vi "Acquisition.vi"(7 "CSM Name":string="CSM-Module") -> ()   [LabVIEW 2026, in "UI-湿度测量.lvlib" / "Acquisition.lvlib"]
doc: "------------- lvcsm -------------\n[CSMStates]\nItem 0 = \"Idle\"\nItem 1 = \"CSM Documentation\"\nItem 2 = \"VI Reference\"\nItem 3 = \"Error Handler\"\nItem 4 = \"Critical Error\"\nItem 5 = \"Target Timeout Error\"\nItem 6 = \"Target Error\"\nItem 7 = \"Async Response\"\nItem 8 = \"Response\"\nItem 9 = \"Async Message Posted\"\nItem 10 = \"Initialize Core Data\"\nItem 11 = \"Exit\"\nItem 12 = \"Data: Initialize\"\nItem 13 = \"Data: Update Indicators\"\nItem 14 = \"Data: Cleanup\"\nItem 15 = \"Macro: Initialize\"\nItem 16 = \"Macro: Exit\"\nItem 17 = \"API: API1\"\nItem 18 = \"API: Start\"\nItem 19 = \"API: Stop\"\nItem 20 = \"DAQ: Initialize\"\nItem 21 = \"DAQ: Acquisite\"\nItem 22 = \"DAQ: Stop\"\nItem 23 = \"DAQ: Close\"\nItem 24 = \"Continuous Check\"\nItem 25 = \"Break Continuous\"\n\n[CSMStatus]\nItem 0 = \"Error Occurred@Error Handler\"\nItem 1 = \"Acquired Data@DAQ: Acquisite\""
uses:
  Acquisition.lvlib
  Supports/Sample Settings.ctl
  Supports/Acquiring States.ctl
  Data ColndSave/Supports/Time and Data.ctl
  13cb97ba-6c5d-4c34-b6e1-a30149b67593.vi
  743750a1-4525-4ef4-b560-e15176358fb5.vi
  0392c9e0-fa12-4efc-b600-051e1718204e.vi
  <userlib>/_NEVSTOP/Communicable State Machine(CSM)/AdvanceAPI/CSM - Revert Arguments-Safe String.vi
  <userlib>/_NEVSTOP/Communicable State Machine(CSM)/_Shared/Trim Single-line Text.vi
  <userlib>/_NEVSTOP/Communicable State Machine(CSM)/AdvanceAPI/CSM - Make String Arguments Safe.vi
  <userlib>/_NEVSTOP/Communicable State Machine(CSM)/AdvanceAPI/CSM - Break Down Multiple States String.vi
  <userlib>/_NEVSTOP/Communicable State Machine(CSM)/AdvanceAPI/CSM - Compact Multiple States.vi
  <userlib>/_NEVSTOP/Communicable State Machine(CSM)/AdvanceAPI/CSM - Keywords.vi
  <userlib>/_NEVSTOP/Communicable State Machine(CSM)/addons/API-String-Arugments-Support/_Support/Convert API String Arguments to Data(variant).vi
  <vilib>/Instr/_visa.llb/VISA Configure Serial Port (Instr).vi
  <userlib>/_NEVSTOP/Communicable State Machine(CSM)/addons/MassData-Parameter/_support/FGV-MassData(lvlibp).vi
  <userlib>/_NEVSTOP/Communicable State Machine(CSM)/Communicable State Machine.lvlib
  <userlib>/_NEVSTOP/Communicable State Machine(CSM)/addons/Loop-Support/CSM Loop Support.lvlib
  Data ColndSave/Data Collection and Save.lvlib
panel:
  out "Error Occurred":errorcluster
  out "State History":string
  in  "Exit":bool
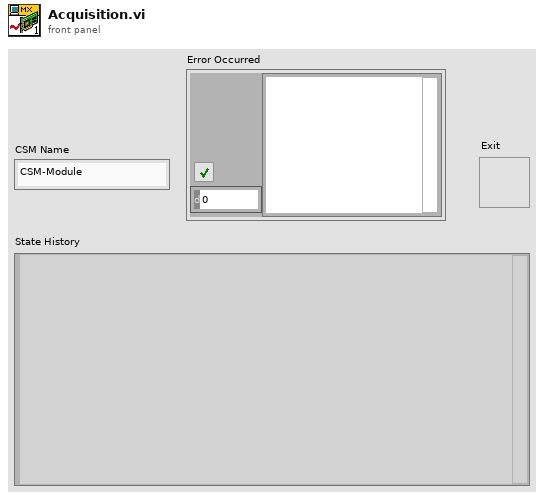
[diagram p1: front panel]
types:
  T1 = enum32{"Invalid", "Standard", "Closed", "Hidden", "Minimized", "Maximized"}
  T2 = enum32{"invalid app kind", "Development System", "Run Time System", "Student Edition", "Embedded LabVIEW", "Evaluation", "Custom"}
  T3 = typedef "UI-湿度测量.lvlib/Acquisition.lvlib/Acquiring States.ctl" = enum16{"Idle", "Acquiring", "Error"}
  T4 = cluster{"波特率":u32, "数据位":u16, "校验":enum16{"None", "Odd", "Even", "Mark", "Space"}, "停止位":u16, "流控制":u16}
  T5 = typedef "Communicable State Machine.lvlib/_CSM_Response Source Message.ctl" = cluster{"‘State":string, "’Arguments":string, "’Error":errorcluster}
  T6 = cluster{"Current VI Reference":refnum<vi>, "Close Panel on Exit?":bool}
  T7 = typedef "UI-湿度测量.lvlib/Sample Settings.ctl" = cluster{"USB Port":refnum<visa-resource-name>, "Interval(s)":dbl}
  T8 = cluster{"Core":cluster{"Current VI Reference":refnum<vi>, "Close Panel on Exit?":bool}, "State":T3, "Sample Settings":T7, "采集时间":timestamp}
  T9 = typedef "Data Collection and Save.lvlib/Time and Data.ctl" = cluster{"采集时间":timestamp, "Data":dbl[]}
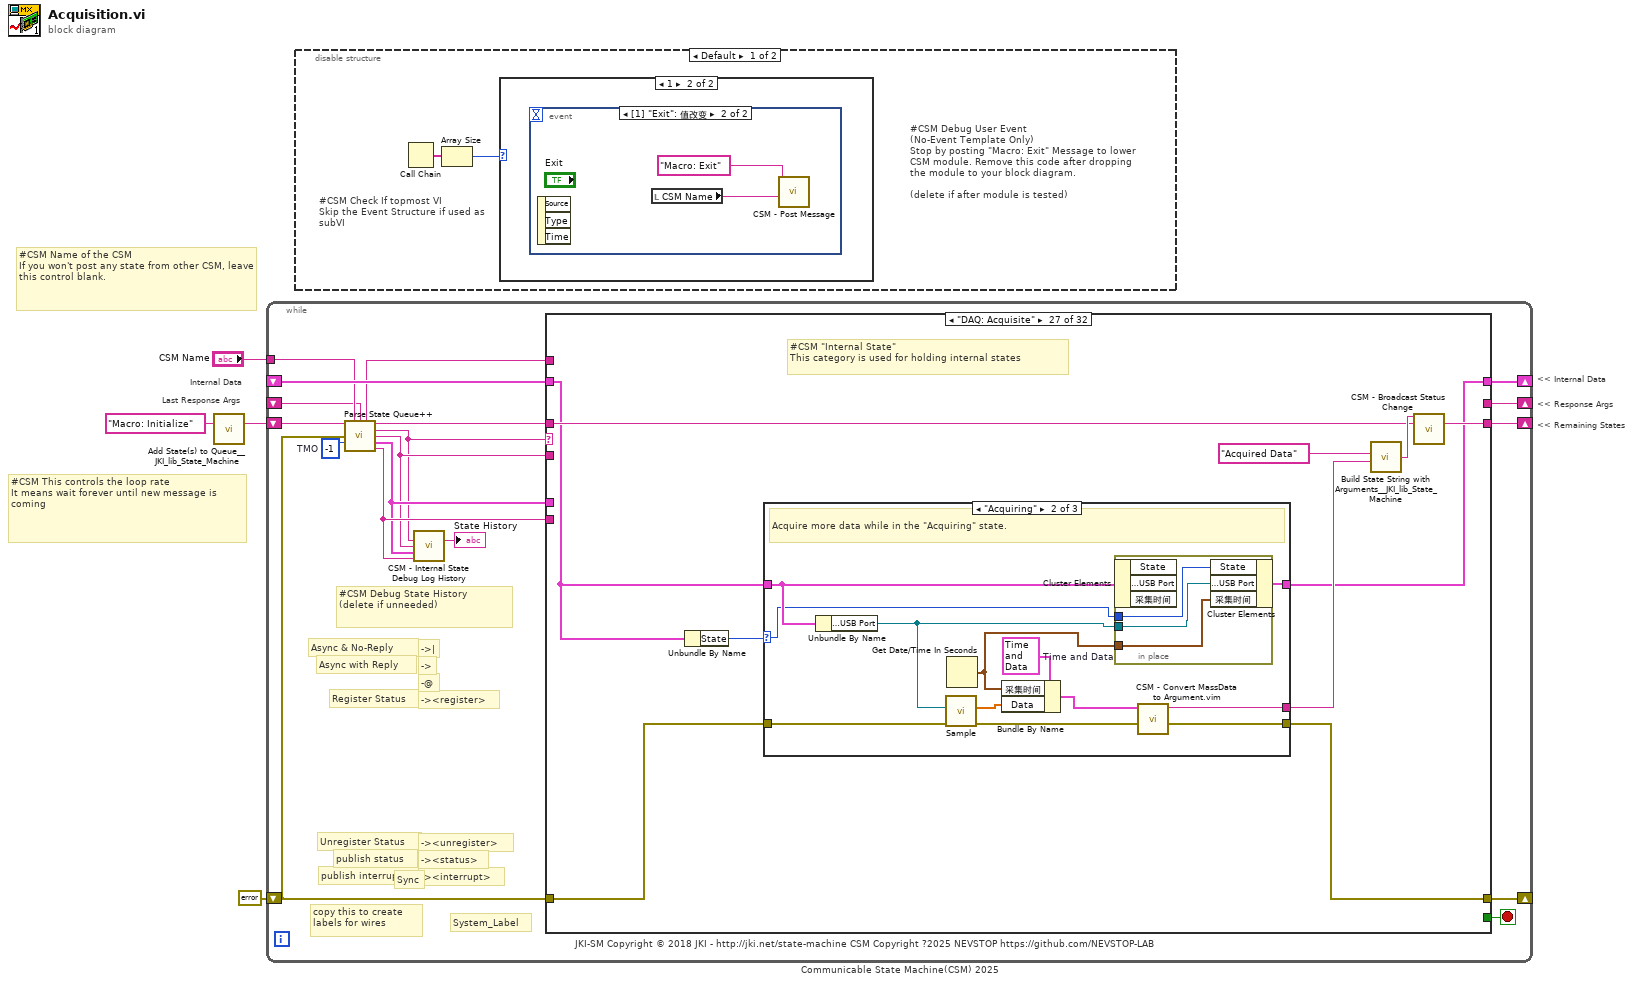
[diagram p0: block diagram]
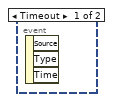
[diagram p3: hidden frame]
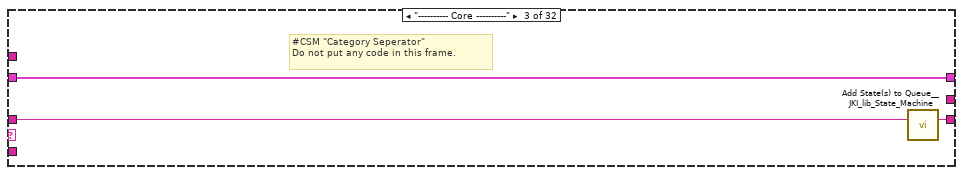
[diagram p7: hidden frame]
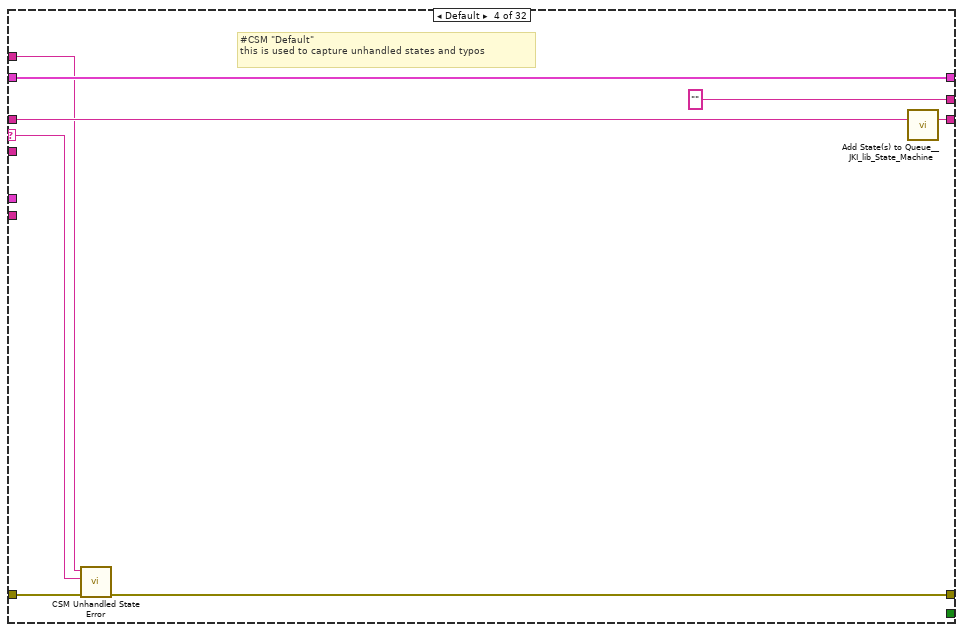
[diagram p8: hidden frame]
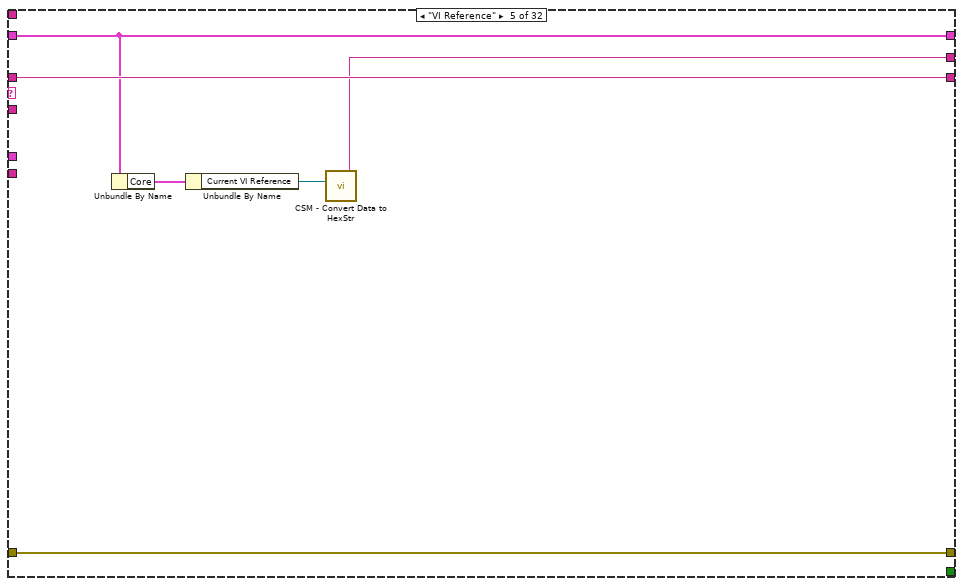
[diagram p9: hidden frame]
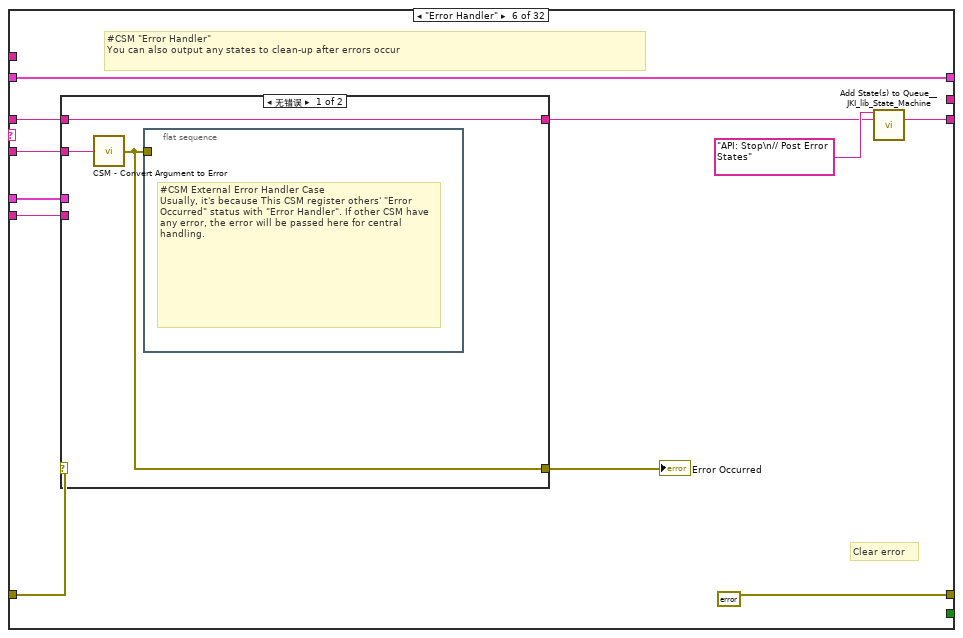
[diagram p10: hidden frame]
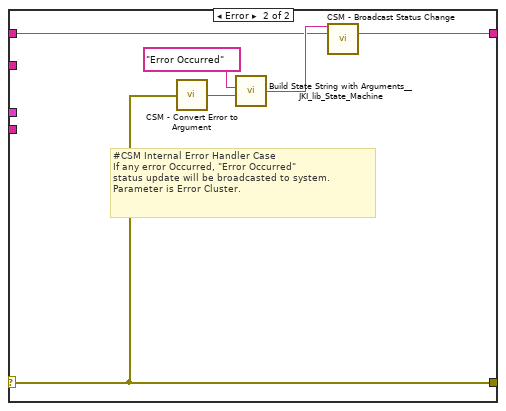
[diagram p11: hidden frame]
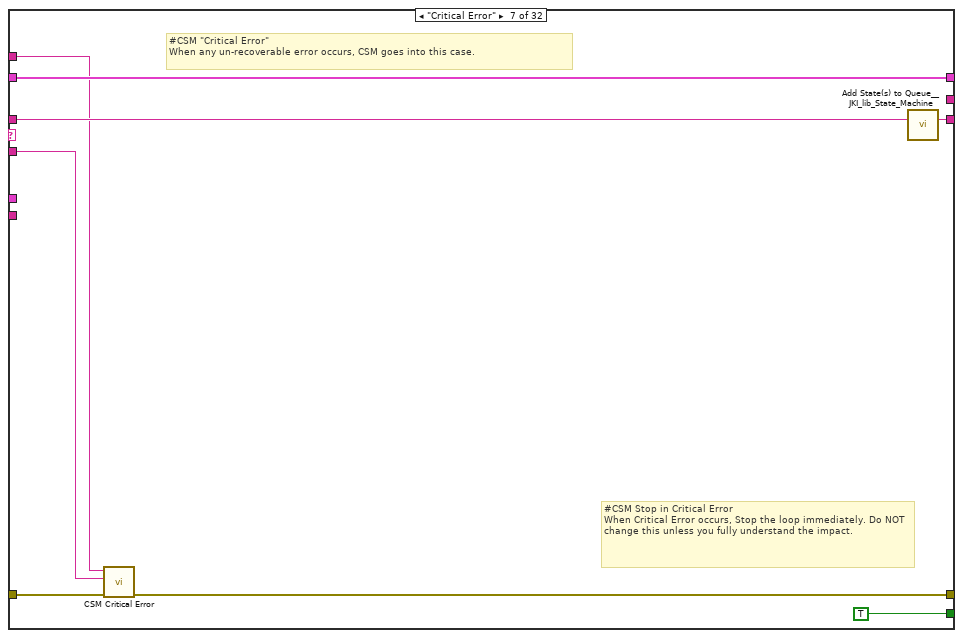
[diagram p12: hidden frame]
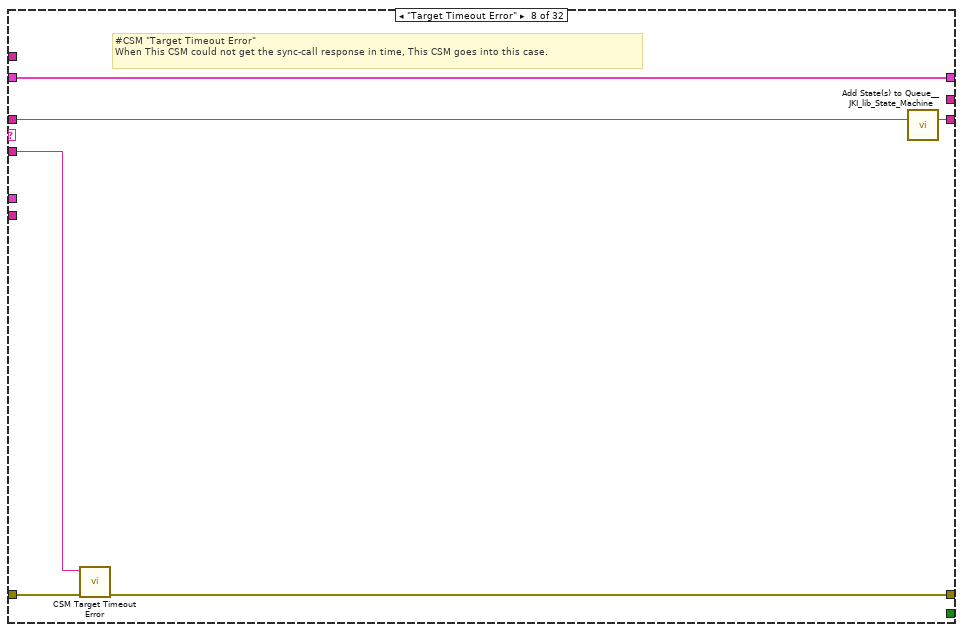
[diagram p13: hidden frame]
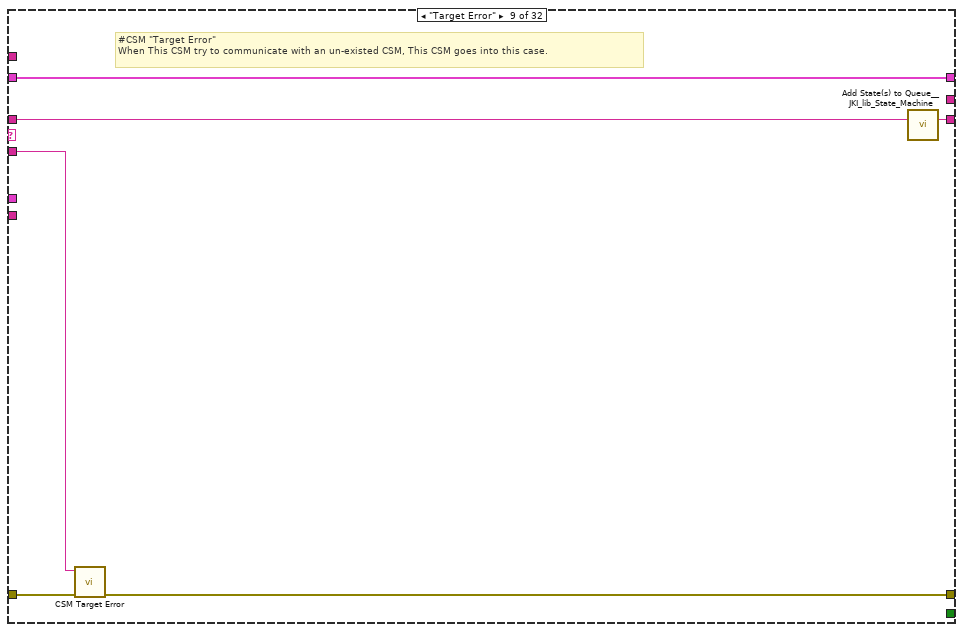
[diagram p14: hidden frame]
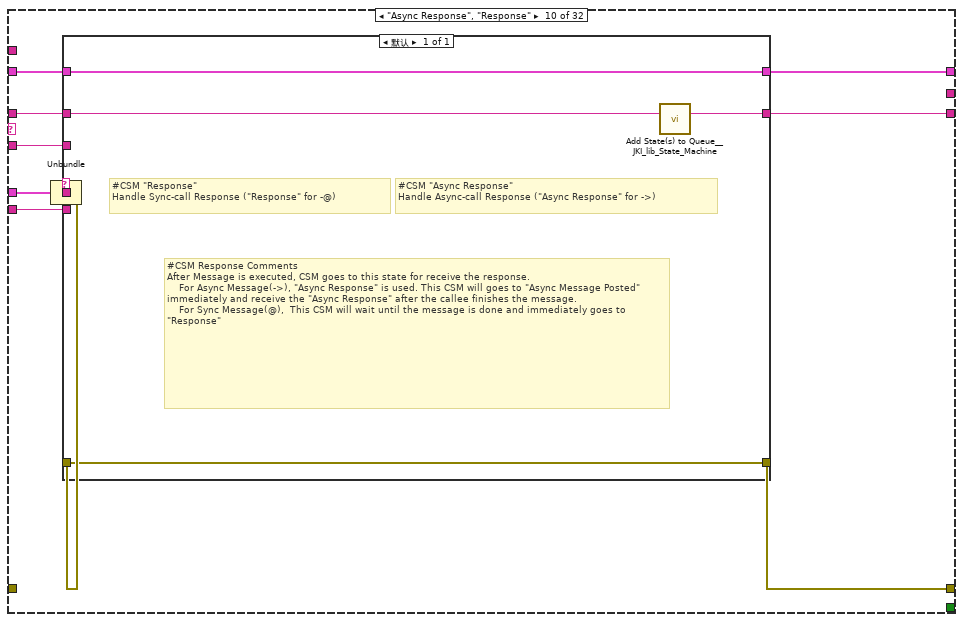
[diagram p15: hidden frame]
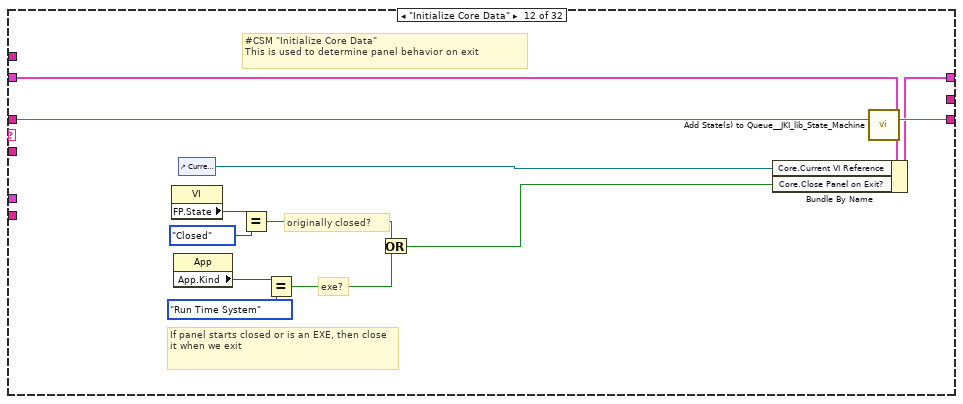
[diagram p17: hidden frame]
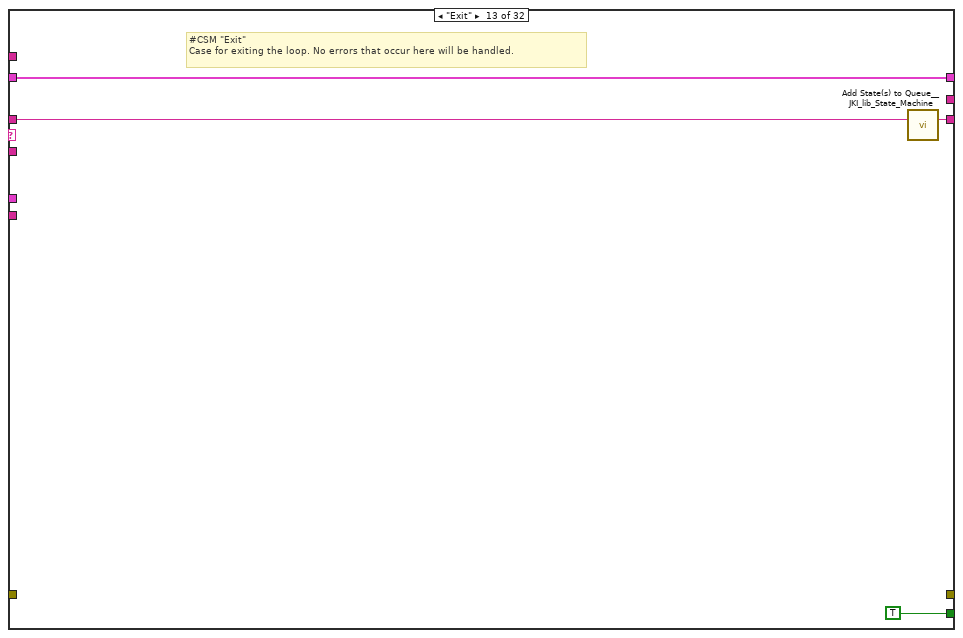
[diagram p18: hidden frame]
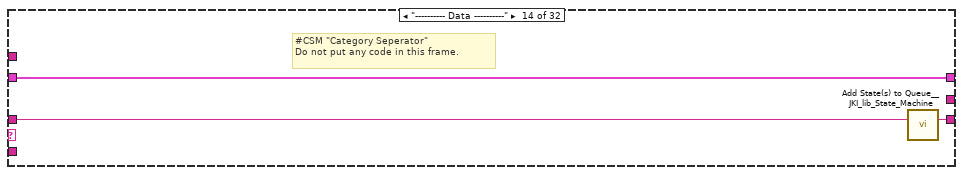
[diagram p19: hidden frame]
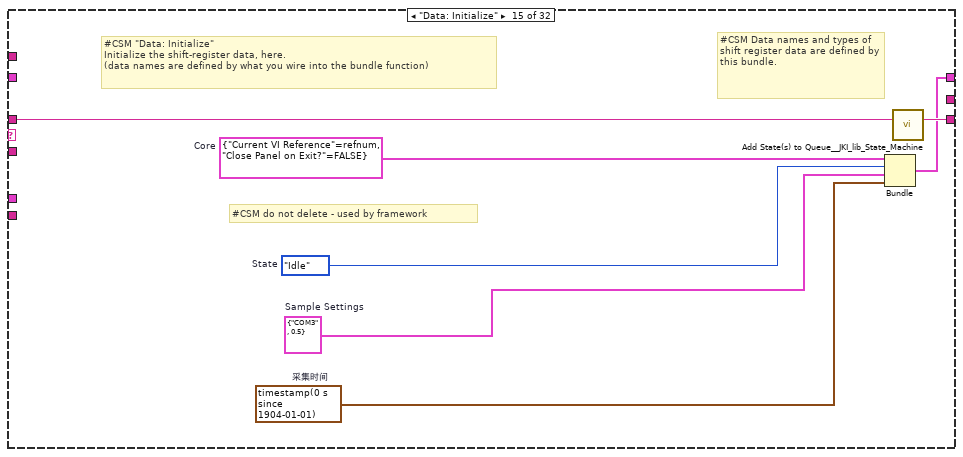
[diagram p20: hidden frame]
diagram:
  # "Last Response Args"
  # "Internal Data"
  # "#CSM Name of the CSM\nIf you won't post any state from other CSM, leave this control blank."
  # "#CSM This controls the loop rate\nIt means wait forever until new message is coming"
  # "<< Internal Data"
  # "<< Response Args"
  # "<< Remaining States"
  n1 = call <vilib>:"Add State(s) to Queue__JKI_lib_State_Machine.vi"("State(s) in (\"\")"="Macro: Initialize" ("Init State(\"Macro: Initialize\")")) -> ("States Out"=w1:string)  [unwired: 14 in]
  n2 = while "Communicable State Machine(CSM) 2025" {
    shift-right: [w17] -> _
    shift-left: _ -> [w16]
    shift-right: [w20] -> _
    shift-left: errorcluster {"status"=FALSE, "code"=0, "source"=""} ("error out") -> [w6]
    shift-right: [w19] -> _
    shift-left: w1 -> [w21]
    tunnel: "CSM Name" -> [w13]
    shift-right: [w14] -> _
    shift-left: _ -> [w8]
    stop <- w18 stop-if-true
    w15 = -1  # TMO
    # "#CSM Debug State History\n(delete if unneeded)"
    # "-><interrupt>"
    # "-><status>"
    # "-><unregister>"
    # "-><register>"
    # "-@"
    # "->"
    # "->|"
    # "publish interrupt"
    # "publish status"
    # "Unregister Status"
    # "Register Status"
    # "Sync"
    # "Async with Reply"
    # "Async & No-Reply"
    # "JKI-SM Copyright © 2018 JKI - http://jki.net/state-machine CSM Copyright ?2025 NEVSTOP https://github.com/NEVSTOP-LAB"
    # "copy this to create labels for wires"
    # "System_Label"
    n3 = call <userlib>:"Parse State Queue++.vi"("State Queue"=w21, "Name (\"\" to Use UUID)"=w13, "Response Arguments"=w8, "Previous Error"=w6, "Dequeue (1 ms)"=w15) -> ("Name Used"=w7:string, "Remaining States"=w22:string, "Current State"=w9:string, "Arguments"=w10:string, "Additional Information"=w11:T5, "Source CSM"=w12:string)  [unwired: 5 in]
    n4 = call <userlib>:"CSM - Internal State Debug Log History.vi"("State"=w9, "Arguments (\"\")"=w10, ">> Response Source Message >>"=w11, "Source (\"\")"=w12) -> ("Debug Log"=→"State History":string)  [unwired: 11 in]
    n5 = case shown="\"DAQ: Acquisite\"" w9 {
      selector: w9 -> [_ _ _ w33 _ _ _ _ _ _ _ _ _ _ _ _ _ _ _ _ _ _ _ _ _ _ _ _ _ _ w251 _]
      tunnel: w22 -> [w23 w26 w29 w37 w42 w48 w71 w77 w83 w93 w100 w112 w116 w119 w126 w129 w135 w138 w142 w150 w155 w162 w174 w184 w188 w201 w208 w233 w239 w242 w252 w257]
      tunnel: w10 -> [_ _ _ _ _ w47 w67 w74 w80 w87 _ _ _ _ _ _ _ _ _ _ _ w159 _ w182 _ _ _ _ _ _ w249 _]
      tunnel: w16 -> [w24 w25 w27 w35 w41 w53 w69 w75 w81 w91 w99 w106 w114 w117 _ w128 w130 w136 w140 w146 w156 w164 w175 w183 w186 w190 w202 w231 w236 w240 w248 w256]
      tunnel: [_ _ _ w30 w43 errorcluster {"status"=FALSE, "code"=0, "source"=""} ("error out") w64 w72 w78 w94 _ _ _ _ _ _ w131 _ _ _ _ _ _ w185 _ w193 w204 _ _ _ _ w258] -> w20
      tunnel: w6 -> [_ _ _ w31 w43 w51 w65 w73 w79 _ _ _ _ _ _ _ w132 _ _ _ _ _ _ w185 _ _ w205 _ _ _ _ w258]
      tunnel: [w23 w26 w28 w36 w42 w49 w70 w76 w82 w92 w100 w111 w115 w118 w125 w129 w134 w137 w141 w149 w154 w161 w173 w184 w187 w201 w207 w232 w238 w241 w250 w255] -> w19
      tunnel: [_ _ _ _ _ _ TRUE _ _ _ _ _ TRUE _ _ _ _ _ _ _ _ _ _ _ _ _ _ _ _ _ _ _] -> w18
      tunnel: [w24 w25 w27 w35 w41 w53 w69 w75 w81 w90 w99 w110 w114 w117 w124 w128 w130 w136 w140 w146 w156 w163 w175 w179 w186 w191 w203 w231 w235 w240 w248 w256] -> w17
      tunnel: w12 -> [_ _ _ _ _ w46 _ _ _ w88 _ _ _ _ _ _ _ _ _ _ _ _ _ _ _ _ _ _ _ _ _ _]
      tunnel: w11 -> [_ _ _ _ _ w45 _ _ _ w89 _ _ _ _ _ _ _ _ _ _ _ _ _ _ _ _ _ _ _ _ _ _]
      tunnel: [_ _ _ "" w38 _ _ _ _ _ _ _ _ _ _ _ _ _ _ _ _ _ _ _ _ _ _ _ _ _ _ _] -> w14
      tunnel: w7 -> [_ _ _ w32 _ _ w66 _ _ _ _ _ _ _ _ _ _ _ _ _ _ _ _ _ _ _ _ _ _ _ _ _]
      frame "", "Idle" {
        # "#CSM \"Idle/Event Handler\"\nexecutes when the state queue is empty"
      }
      frame "CSM Documentation" {
        # "#CSM State Syntax\n\n// Comment line, all text to the right of “//” will be ignored\n// Local Message Example\nDoSth: DoA >> Arguments\n\n// Sync Call Example\nAPI: xxxx >> Arguments -@ TargetModule\n\n// Async Call Example\nAPI: xxxx >> Arguments -> TargetModule\n\n// Async Call without Reply Example\nAPI: xxxx >> Arguments ->| TargetModule\n\n// Broadcast normal status:\nStatus >> StatusArguments  -><status>\n\n// Broadcast Interrupt status:\nInterrupt >> StatusArguments  -><interrupt>\n\n// Register Source Module's status to Handler Module\nStatus@Source Module >> Handler Module@Handler Module -><register>\n\n// Unegister Source Module's status\nStatus@Source Module >> Handler Module -><unregister>"
        # "#CSM README FIRST\n\nCommunicable State Machine(CSM) is a LabVIEW application framework that builds upon JKI State Machine(JKISM). It follows the pattern of JKISM and extends the keywords to describe message communication between modules, including concepts such as Sync-Message, Async-Message, Subscription/Unsubscription of status - essential elements for creating reusable code modules. For more information, please visit the CSM wiki: https://nevstop-lab.github.io/CSM-Wiki/\n\nFor instructions on JKI State Machine, visit: \n    http://jki.net/state-machine/\nFor information about CSM, visit: \n    https://github.com/NEVSTOP-LAB"
        # "#CSM \"Documentation\"\nCase for holding CSM Documenation"
      }
      frame "---------- Core ----------" {
        # "#CSM \"Category Seperator\"\nDo not put any code in this frame."
        n6 = call <vilib>:"Add State(s) to Queue__JKI_lib_State_Machine.vi"("State(s) in (\"\")"=w29) -> ("States Out"=w28:string)  [unwired: 14 in]
      }
      frame Default {
        # "#CSM \"Default\"\nthis is used to capture unhandled states and typos"
        n7 = call <userlib>:"CSM Unhandled State Error.vi"("error in (no error)"=w31, "Undefined State"=w33, "CSM Name"=w32) -> ("error out"=w30:errorcluster)  [unwired: 8 in]
        n8 = call <vilib>:"Add State(s) to Queue__JKI_lib_State_Machine.vi"("State(s) in (\"\")"=w37) -> ("States Out"=w36:string)  [unwired: 14 in]
      }
      frame "VI Reference" {
        n9 = Unbundle By Name(w41) -> ("Core"=w40:T6)
        n10 = Unbundle By Name(w40) -> ("Current VI Reference"=w39:refnum<vi>)
        n11 = call <userlib>:"CSM - Convert Data to HexStr.vi"("Variant"=w39) -> ("HEX String (0-9,A-F)"=w38:string)  [unwired: 8 in]
      }
      frame "Error Handler" {
        # "#CSM \"Error Handler\"\nYou can also output any states to clean-up after errors occur"
        # "Clear error"
        n12 = case shown="无错误" w51 {
          selector: w51 -> [_ w58]
          tunnel: [w57 w60] -> w50
          tunnel: w48 -> [w57 w59]
          tunnel: w47 -> [w56 _]
          tunnel: w46 -> [_ _]
          tunnel: w45 -> [_ _]
          tunnel: [w55 w58] -> w44
          frame No Error {
            n13 = call <userlib>:"CSM - Convert Argument to Error.vi"("Argument"=w56) -> ("Error"=w55:errorcluster)  [unwired: 4 in]
            n14 = flat-sequence {
              tunnel: w55 -> [_]
              frame #0 {
                # "#CSM External Error Handler Case\nUsually, it's because This CSM register others' \"Error Occurred\" status with \"Error Handler\". If other CSM have any error, the error will be passed here for central handling."
              }
            }
          }
          frame Error {
            # "#CSM Internal Error Handler Case \nIf any error Occurred, \"Error Occurred\" \nstatus update will be broadcasted to system.\nParameter is Error Cluster."
            n15 = call <userlib>:"CSM - Convert Error to Argument.vi"("Error"=w58) -> ("Argument"=w62:string)  [unwired: 4 in]
            n16 = call <vilib>:"Build State String with Arguments__JKI_lib_State_Machine.vi"("Arguments (\"\")"=w62, "State"="Error Occurred" ("Status with Arguments")) -> ("State with Arguments"=w61:string)  [unwired: 4 in]
            n17 = call <userlib>:"CSM - Broadcast Status Change.vi"("Status With Arguments"=w61, "State Queue"=w59) -> ("Remaining States"=w60:string)  [unwired: 13 in]
          }
        }
        "Error Occurred" <- w44
        n18 = call <vilib>:"Add State(s) to Queue__JKI_lib_State_Machine.vi"("State(s) in Front (\"\")"="API: Stop\n// Post Error States", "State(s) in (\"\")"=w50) -> ("States Out"=w49:string)  [unwired: 13 in]
      }
      frame "Critical Error" {
        # "#CSM \"Critical Error\"\nWhen any un-recoverable error occurs, CSM goes into this case."
        # "#CSM Stop in Critical Error\nWhen Critical Error occurs, Stop the loop immediately. Do NOT change this unless you fully understand the impact."
        n19 = call <userlib>:"CSM Critical Error.vi"("error in (no error)"=w65, "Arugments (As Reason)"=w67, "CSM Name"=w66) -> ("error out"=w64:errorcluster)  [unwired: 8 in]
        n20 = call <vilib>:"Add State(s) to Queue__JKI_lib_State_Machine.vi"("State(s) in (\"\")"=w71) -> ("States Out"=w70:string)  [unwired: 14 in]
      }
      frame "Target Timeout Error" {
        # "#CSM \"Target Timeout Error\"\nWhen This CSM could not get the sync-call response in time, This CSM goes into this case."
        n21 = call <userlib>:"CSM Target Timeout Error.vi"("error in (no error)"=w73, "Arguments (As CSM Name)"=w74) -> ("error out"=w72:errorcluster)  [unwired: 9 in]
        n22 = call <vilib>:"Add State(s) to Queue__JKI_lib_State_Machine.vi"("State(s) in (\"\")"=w77) -> ("States Out"=w76:string)  [unwired: 14 in]
      }
      frame "Target Error" {
        # "#CSM \"Target Error\"\nWhen This CSM try to communicate with an un-existed CSM, This CSM goes into this case."
        n23 = call <userlib>:"CSM Target Error.vi"("error in (no error)"=w79, "Arguments (As CSM Name)"=w80) -> ("error out"=w78:errorcluster)  [unwired: 9 in]
        n24 = call <vilib>:"Add State(s) to Queue__JKI_lib_State_Machine.vi"("State(s) in (\"\")"=w83) -> ("States Out"=w82:string)  [unwired: 14 in]
      }
      frame "Async Response", "Response" {
        n25 = Unbundle(w89) -> ("‘State"=w86:string, "’Arguments"=w85:string, "’Error"=w84:errorcluster)
        n26 = case shown="默认" w86 {
          tunnel: [w95] -> w92
          tunnel: w93 -> [w96]
          tunnel: [w98] -> w90
          tunnel: w91 -> [w98]
          tunnel: [w97] -> w94
          tunnel: w84 -> [w97]
          tunnel: w88 -> [_]
          tunnel: w87 -> [_]
          tunnel: w85 -> [_]
          frame 默认 {
            # "#CSM \"Async Response\"\nHandle Async-call Response (\"Async Response\" for ->)"
            # "#CSM \"Response\"\nHandle Sync-call Response (\"Response\" for -@)"
            # "#CSM Response Comments\nAfter Message is executed, CSM goes to this state for receive the response.\n    For Async Message(->), \"Async Response\" is used. This CSM will goes to \"Async Message Posted\" immediately and receive the \"Async Response\" after the callee finishes the message.\n    For Sync Message(@),  This CSM will wait until the message is done and immediately goes to \"Response\""
            n27 = call <vilib>:"Add State(s) to Queue__JKI_lib_State_Machine.vi"("State(s) in (\"\")"=w96) -> ("States Out"=w95:string)  [unwired: 14 in]
          }
        }
      }
      frame "Async Message Posted" {
        # "#CSM \"Async Message Posted\"\nAfter Async Message is posted (-> or ->| ), CSM goes to this state for post-action.\nYou can use Argument - State to tell which Async Message is called."
      }
      frame "Initialize Core Data" {
        # "#CSM \"Initialize Core Data\"\nThis is used to determine panel behavior on exit"
        # "originally closed?"
        # "exe?"
        # "If panel starts closed or is an EXE, then close it when we exit"
        n28 = property class="VI"() -> ("FP.State"=w103:T1)  [unwired: 2 in, 2 out]
        n29 = property class="App"() -> ("App.Kind"=w109:T2)  [unwired: 2 in, 2 out]
        n30 = control-ref of="Current VI Reference"() -> (w104:refnum<vi>)
        n31 = Equal?(x=w103, y=T1."Closed" ("Front Panel Window:State")) -> (x = y?=w101:bool)
        n32 = Equal?(x=w109, y=T2."Run Time System" ("Application:Kind")) -> (x = y?=w107:bool)
        n33 = Or(x=w101, y=w107) -> (x .or. y?=w105:bool)
        n34 = Bundle By Name(cluster=w106, "Core.Current VI Reference"=w104, "Core.Close Panel on Exit?"=w105) -> (w110:T8)
        n35 = call <vilib>:"Add State(s) to Queue__JKI_lib_State_Machine.vi"("State(s) in (\"\")"=w112) -> ("States Out"=w111:string)  [unwired: 14 in]
      }
      frame "Exit" {
        # "#CSM \"Exit\"\nCase for exiting the loop. No errors that occur here will be handled."
        n36 = call <vilib>:"Add State(s) to Queue__JKI_lib_State_Machine.vi"("State(s) in (\"\")"=w116) -> ("States Out"=w115:string)  [unwired: 14 in]
      }
      frame "---------- Data ----------" {
        # "#CSM \"Category Seperator\"\nDo not put any code in this frame."
        n37 = call <vilib>:"Add State(s) to Queue__JKI_lib_State_Machine.vi"("State(s) in (\"\")"=w119) -> ("States Out"=w118:string)  [unwired: 14 in]
      }
      frame "Data: Initialize" {
        w120 = timestamp(0 s since 1904-01-01)  # 采集时间
        w121 = Acquiring_States."Idle"  # State
        w122 = T7 {"USB Port"="COM3", "Interval(s)"=0.5}  # Sample Settings
        w123 = T6 {"Current VI Reference"=refnum, "Close Panel on Exit?"=FALSE}  # Core
        # "#CSM \"Data: Initialize\"\nInitialize the shift-register data, here.\n(data names are defined by what you wire into the bundle function)"
        # "#CSM do not delete - used by framework"
        # "#CSM Data names and types of shift register data are defined by this bundle."
        n38 = Bundle("Core"=w123, "State"=w121, "Sample Settings"=w122, "采集时间"=w120) -> (w124:T8)  [unwired: 1 in]
        n39 = call <vilib>:"Add State(s) to Queue__JKI_lib_State_Machine.vi"("State(s) in (\"\")"=w126) -> ("States Out"=w125:string)  [unwired: 14 in]
      }
      frame "Data: Update Indicators" {
        n40 = local write "Error Occurred"(errorcluster {"status"=FALSE, "code"=0, "source"=""} ("错误常量")) -> ()
      }
      frame "Data: Cleanup" {
        # "#CSM \"Data: Cleanup\"\nCleanup any data and references, here.\n(this is called automatically, by the Macro: Exit)"
        n41 = Unbundle By Name(w130) -> ("Core.Current VI Reference"=w133:refnum<vi>)
        n42 = Close Reference(reference=w133, error in (no error)=w132) -> (error out=w131:errorcluster)
        n43 = call <vilib>:"Add State(s) to Queue__JKI_lib_State_Machine.vi"("State(s) in (\"\")"=w135) -> ("States Out"=w134:string)  [unwired: 14 in]
      }
      frame "---------- Macro ----------" {
        # "#CSM \"Category Seperator\"\nDo not put any code in this frame."
        n44 = call <vilib>:"Add State(s) to Queue__JKI_lib_State_Machine.vi"("State(s) in (\"\")"=w138) -> ("States Out"=w137:string)  [unwired: 14 in]
      }
      frame "Macro: Initialize" {
        # "#CSM \"Macro: Initialize\"\nInitialization Macro (This is called once, when the VI starts)"
        n45 = call <vilib>:"Add State(s) to Queue__JKI_lib_State_Machine.vi"("State(s) in Front (\"\")"="Data: Initialize\nInitialize Core Data\nData: Update Indicators", "State(s) in (\"\")"=w142) -> ("States Out"=w141:string)  [unwired: 13 in]
      }
      frame "Macro: Exit" {
        # "#CSM \"Macro: Exit\"\nExit Macro (This is called once, when the VI exits)"
        n46 = Unbundle By Name(w146) -> ("State"=w145:T3)
        n47 = case shown="\"Acquiring\"" w145 {
          tunnel: ["" "Break Continuous\nDAQ: Close" ""] -> w143
          frame "Idle", Default {
          }
          frame "Acquiring" {
          }
          frame "Error" {
          }
        }
        n48 = call <vilib>:"Add State(s) to Queue__JKI_lib_State_Machine.vi"("State(s) in Front (\"\")"="//Exit Sub-Modules ", "State(s) in (\"\")"=w143, "State(s) at Back (\"\")"="Data: Cleanup\nExit") -> ("States Out"=w147:string)  [unwired: 12 in]
        n49 = call <vilib>:"Add State(s) to Queue__JKI_lib_State_Machine.vi"("State(s) in Front (\"\")"=w147, "State(s) in (\"\")"=w150) -> ("States Out"=w149:string)  [unwired: 13 in]
      }
      frame "---------- API ----------" {
        # "#CSM \"Category Seperator\"\nDo not put any code in this frame."
        n50 = call <vilib>:"Add State(s) to Queue__JKI_lib_State_Machine.vi"("State(s) in (\"\")"=w155) -> ("States Out"=w154:string)  [unwired: 14 in]
      }
      frame "API: Start" {
        w158 = T7 {"USB Port"="COM3", "Interval(s)"=0.5}  # Sample Settings
        # "#CSM-NOTE\nhttps://github.com/NEVSTOP-LAB/CSM-Continuous-Meausrement-and-Logging/issues/21\n\nUse CSM-Loop Support to define a loop in CSM, which is recommanded."
        # "#CSM API Example\nCopy/Rename this case for your own API"
        n51 = Unbundle By Name(w164) -> ("State"=w166:T3)
        n52 = case shown="\"Idle\"" w166 {
          selector: w166 -> [_ w170 w171]
          tunnel: [Acquiring_States."Acquiring" ("Acquisition State") w170 w171] -> w167
          tunnel: ["DAQ: Initialize \nDAQ: Acquisite\nContinuous Check >> DAQ: Acquisite -><loop> \nDAQ: Stop\nDAQ: Close " ("State(s) in Front (\"\")") _ _] -> w165
          frame "Idle" {
            # "If the system is idle, start the acquisition."
          }
          frame "Acquiring" {
            # "The system is already acquiring. Ignore the \"Start\" message."
          }
          frame "Error" {
          }
        }
        n53 = local write "Error Occurred"(errorcluster {"status"=FALSE, "code"=0, "source"=""} ("错误常量")) -> ()
        n54 = call "Convert API String Arguments to Data.vim"("Reference Type"=w158, "API String"=w159) -> ("Data"=w157:T7)  [unwired: 6 in, 1 out]
        n55 = call <userlib>:"CSMLS - Define Loop State(s).vi"("Loop States"=w165, "States Queue"=w162) -> ("Remaining States"=w161:string)  [unwired: 13 in]
        n56 = Bundle By Name(cluster=w164, "State"=w167, "Sample Settings"=w157) -> (w163:T8)
      }
      frame "API: Stop" {
        # "#CSM API Example\nCopy/Rename this case for your own API"
        n57 = Unbundle By Name(w175) -> ("State"=w176:T3)
        n58 = case shown="\"Acquiring\"" w176 {
          tunnel: [_ "Break Continuous" ("State(s) in Front (\"\")") "Break Continuous" ("State(s) in Front (\"\")")] -> w172
          frame "Idle" {
            # "The system is already idle. Ignore the \"Stop\" message."
          }
          frame "Acquiring" {
            # "If the system is acquiring, stop the acquisition."
          }
          frame "Error" {
          }
        }
        n59 = call <vilib>:"Add State(s) to Queue__JKI_lib_State_Machine.vi"("State(s) in Front (\"\")"=w172, "State(s) in (\"\")"=w174) -> ("States Out"=w173:string)  [unwired: 13 in]
      }
      frame "API: Sample Interval" {
        n60 = call "Convert API String Arguments to Data.vim"("Reference Type"=0.0, "API String"=w182) -> ("Data"=w180:dbl)  [unwired: 6 in, 1 out]
        n61 = Bundle By Name(cluster=w183, "Sample Settings.Interval(s)"=w180) -> (w179:T8)
      }
      frame "---------- DAQ ----------" {
        # "#CSM \"Category Seperator\"\nDo not put any code in this frame."
        n62 = call <vilib>:"Add State(s) to Queue__JKI_lib_State_Machine.vi"("State(s) in (\"\")"=w188) -> ("States Out"=w187:string)  [unwired: 14 in]
      }
      frame "DAQ: Initialize" {
        # "#CSM \"Category Seperator\"\nDo not put any code in this frame."
        n63 = Unbundle By Name(w190) -> ("Sample Settings.USB Port"=w189:refnum<visa-resource-name>)
        n64 = Unbundle By Name(T4 {"波特率"=9600, "数据位"=8, "校验"=enum."None", "停止位"=10, "流控制"=0} ("串口设置")) -> ("波特率"=w196:u32, "数据位"=w197:u16, "校验"=w198:enum16{"None", "Odd", "Even", "Mark", "Space"}, "停止位"=w199:u16, "流控制"=w200:u16)
        n65 = call-poly "VISA Configure Serial Port"("VISA resource name"=w189, "timeout (10sec)"=u32 3000, "baud rate (9600)"=w196, "data bits (8)"=w197, "parity (0:none)"=w198, "stop bits (10: 1 bit)"=w199, "flow control (0:none)"=w200) -> ("VISA resource name out"=w192:refnum<visa-resource-name>, "error out"=w193:errorcluster)  [unwired: 2 in, 5 out]
        n66 = Bundle By Name(cluster=w190, "Sample Settings.USB Port"=w192) -> (w191:T8)
      }
      frame "DAQ: Acquisite" {
        # "#CSM \"Internal State\"\nThis category is used for holding internal states"
        n67 = Unbundle By Name(w202) -> ("State"=w210:T3)
        n68 = case shown="\"Acquiring\"" w210 {
          selector: w210 -> [_ w216 _]
          tunnel: [w213 w224 w230] -> w204
          tunnel: w205 -> [w213 w223 w230]
          tunnel: [w212 w217 w229] -> w203
          tunnel: w202 -> [w212 w218 w229]
          tunnel: [_ w225 _] -> w206
          frame "Idle" {
            # "Ignore \"Acquire\" messages when the acquisition is idle."
          }
          frame "Acquiring" {
            w221 = T9 {"采集时间"=timestamp(0 s since 1904-01-01), "Data"=[]}  # Time and Data
            # "Acquire more data while in the \"Acquiring\" state."
            n69 = Unbundle By Name(w218) -> ("Sample Settings.USB Port"=w215:refnum<visa-resource-name>)
            n70 = call "Sample.vi"("错误输入（无错误）"=w223, "VISA资源名称"=w215) -> ("error out"=w222:errorcluster, "Data Out"=w220:dbl[])  [unwired: 8 in]
            n71 = Get Date/Time In Seconds() -> (seconds since 1Jan1904=w214:timestamp)
            n72 = Bundle By Name(cluster=w221, "采集时间"=w214, "Data"=w220) -> (w219:T9)
            n73 = in-place {
              in-place-border: w216 -> [w228]
              in-place-border: w214 -> [w227]
              in-place-border: w215 -> [w226]
              n74 = in-place-cluster #1(w218) -> ()  [unwired: 3 out]
              n75 = in-place-cluster #1("State"=w228, "Sample Settings.USB Port"=w226, "采集时间"=w227) -> (w217:T8)
            }
            n76 = call "CSM - Convert MassData to Argument.vim"("error in (no error)"=w222, "Data"=w219) -> ("error out"=w224:errorcluster, "MassData Argument"=w225:string)  [unwired: 6 in]
          }
          frame "Error" {
          }
        }
        n77 = call <vilib>:"Build State String with Arguments__JKI_lib_State_Machine.vi"("Arguments (\"\")"=w206, "State"="Acquired Data" ("Status with Arguments")) -> ("State with Arguments"=w211:string)  [unwired: 4 in]
        n78 = call <userlib>:"CSM - Broadcast Status Change.vi"("Status With Arguments"=w211, "State Queue"=w208) -> ("Remaining States"=w207:string)  [unwired: 13 in]
      }
      frame "DAQ: Stop" {
        # "#CSM \"Internal State\"\nThis category is used for holding internal states"
        n79 = call <vilib>:"Add State(s) to Queue__JKI_lib_State_Machine.vi"("State(s) in (\"\")"=w233) -> ("States Out"=w232:string)  [unwired: 14 in]
      }
      frame "DAQ: Close" {
        w234 = Acquiring_States."Idle"  # State
        # "#CSM \"Internal State\"\nThis category is used for holding internal states"
        n80 = Unbundle By Name(w236) -> ("Sample Settings.USB Port"=w237:refnum<visa-resource-name>)
        n81 = VISA Close(VISA resource name=w237) -> ()  [unwired: 1 in, 1 out]
        n82 = Bundle By Name(cluster=w236, "State"=w234) -> (w235:T8)
        n83 = call <vilib>:"Add State(s) to Queue__JKI_lib_State_Machine.vi"("State(s) in (\"\")"=w239) -> ("States Out"=w238:string)  [unwired: 14 in]
      }
      frame "---------- Loop ----------" {
        # "#CSM \"Internal State\"\nThis category is used for holding internal states"
        n84 = call <vilib>:"Add State(s) to Queue__JKI_lib_State_Machine.vi"("State(s) in (\"\")"=w242) -> ("States Out"=w241:string)  [unwired: 14 in]
      }
      frame "Continuous Check" {
        # "#CSM \"Internal State\"\nThis category is used for holding internal states"
        n85 = Unbundle By Name(w248) -> ("Sample Settings.Interval(s)"=w254:dbl, "采集时间"=w246:timestamp)
        n86 = Get Date/Time In Seconds() -> (seconds since 1Jan1904=w247:timestamp)
        n87 = Multiply(x=u32 1000 ("y"), y=w254) -> (x*y=w245:dbl)
        n88 = Subtract(x=w247, y=w246) -> (x-y=w244:dbl)
        n89 = Subtract(x=w245, y=w244) -> (x-y=w243:dbl)
        n90 = Wait (ms)(milliseconds to wait=w243) -> ()  [unwired: 1 out]
        n91 = call <userlib>:"CSMLS - Append Continuous State.vi"("Loop State(s) And Arguments"=w249, "Continous Arguments (\"\")"=w249, "Continous State"=w251, "States Queue"=w252) -> ("Remaining States"=w250:string)  [unwired: 7 in]
      }
      frame "Break Continuous" {
        n92 = call <userlib>:"CSMLS - Remove Loop Tag to Break.vi"("States Queue"=w257) -> ("Remaining States"=w255:string)  [unwired: 10 in]
      }
    }
  }
  n93 = disable-structure shown="Default" {
    frame condition #0 (active) {
      # "#CSM Check If topmost VI\nSkip the Event Structure if used as subVI"
      # "#CSM Debug User Event\n(No-Event Template Only)\nStop by posting \"Macro: Exit\" Message to lower CSM module. Remove this code after dropping the module to your block diagram. \n\n(delete if after module is tested)"
      n94 = Call Chain() -> (call chain=w260:string[])
      n95 = Array Size(array=w260) -> (size(s)=w259:i32)
      n96 = case shown="1" w259 {
        frame Default {
        }
        frame 1 {
          n97 = event shown="[1] \"Exit\": 值改变" {
            selector: _ -> [_ _]
            dyn-events: _ -> [_ _]
            timeout: _ -> [_ _]
            event Timeout {
              n98 = event-data() -> ()  [unwired: 1 in, 3 out]
            }
            event "Exit": Value Change {
              n99 = event-data() -> ()  [unwired: 1 in, 3 out]
              n100 = local read "CSM Name"() -> (w262:string)
              n101 = call <userlib>:"CSM - Post Message.vi"("Target Module"=w262, "State"="Macro: Exit" ("States")) -> ()  [unwired: 9 in, 1 out]
            }
          }
        }
      }
    }
    frame condition #1 {
    }
  }
